vi "Impedance_Sweep_Freq.vi"(6 "Save Data?":bool, 8 "Freq Info":T1={"type"=1, "Number of\nTest Freqs"=128, "Start Freq"=100.0, "Stop Freq"=50000.0} {"Stop Freq" format="%#.4p"; "Start Freq" format="%#.4p"; "type" items=["Linear", "Logarithmic"]}, 9 "Saving Cluster":T2={"Experiment Title"="Experiment Title", "Save Path"=path "C:/Users/Human-MPI/Desktop/Temp", "File Name String"="TestStats", "Meta-Data Array"=[1.0]}, 10 "LCR Params":T4={"Rg_Vmon"=5000.0, "Rg_Imon"=5000.0, "ESL_Cal"=2.5e-07, "ESR_Cal"=0.0, "Cp_Cal"=0.0, "Rp_Cal"=1000000000.0, "UseCorrection"=TRUE, "R_Shunt"=100.0} {"R_Shunt" format="%#_6p"; "Rg_Vmon" format="%#_6p"; "Rg_Imon" format="%#_6p"; "ESL_Cal" format="%#_6p"; "ESR_Cal" format="%#_6p"; "Cp_Cal" format="%#_6p"; "Rp_Cal" format="%#_6p"}, 11 "Test Params Cluster":T3={"Test Freq. (Hz)"=0.0, "Output Signal Amplitude\nVolts Pk"=0.1, "Sampling Time (s)"=0.1, "Sampling Rate (Hz)"=2000000.0, "Output Channel"="PXI1Slot2/ao1", "Current Channel"="PXI1Slot2/ai1", "Voltage Channel"="PXI1Slot2/ai0", "Trigger Channel"="/PXI1Slot2/ao/StartTrigger", "Number of runs"=5} {"Output Signal Amplitude\nVolts Pk" format="%#_6p"; "Sampling Time (s)" format="%#_6p"; "Sampling Rate (Hz)" format="%#_6p"}) -> (0 "Single Run \nImpedance Cluster":T5={"|Z|"=nan, "Phase(Z)"=nan, "Re(Z)"=nan, "Imag(Z)"=nan, "Ls"=nan, "Cs"=nan, "Rp"=0.0, "Cp"=0.0} {"|Z|" format="%#_5p"; "Phase(Z)" format="%#_5p"; "Re(Z)" format="%#_5p"; "Imag(Z)" format="%#_5p"; "Ls" format="%#_5p"; "Cs" format="%#_5p"; "Rp" format="%#_5p"; "Cp" format="%#_5p"}, 1 "RealImag Graph":cluster{dbl[], dbl[]}[](graph), 2 "Mag Phase Graph":cluster{dbl[], dbl[]}[](graph), 3 "output cluster":T3={"Test Freq. (Hz)"=3243.3070866141734, "Output Signal Amplitude\nVolts Pk"=0.1, "Sampling Time (s)"=0.01, "Sampling Rate (Hz)"=250000.0, "Output Channel"="Dev3/ao0", "Current Channel"="Dev3/ai1", "Voltage Channel"="Dev3/ai0", "Trigger Channel"="/Dev3/ao/StartTrigger", "Number of runs"=5}, 4 "2D Compass":refnum<class "2D Plot Datatype.lvclass">[](xcontrol), 7 "Progress":i32(slide) scale=0.0..100.0)   [LabVIEW 2021]
uses:
  <vilib>/Math Plots/2D Math Plots/2D Compass/2D Compass XCtrl/2D Compass.xctl
  <vilib>/Analysis/1siggen.llb/Ramp Pattern by Samples.vi
  <vilib>/Analysis/baseanly.llb/Mean (DBL).vi
  <vilib>/Math Plots/2D Math Plots/2D Compass/2D Compass Datatype/Public/Plot Helper (Vector).vi
  <vilib>/Analysis/NI_AALBase.lvlib
  <vilib>/Math Plots/2D Math Plots/2D Compass/2D Compass Datatype/2D Compass Datatype.lvclass
panel:
  in  "Tab Control":enum32{"Inputs", "Outputs", "Additional Plots"}(tab)
  out "Test Number":i32=8
  out "Mean Mag":dbl format="%.4p"
  out "Mean Phase":dbl format="%0.2f"
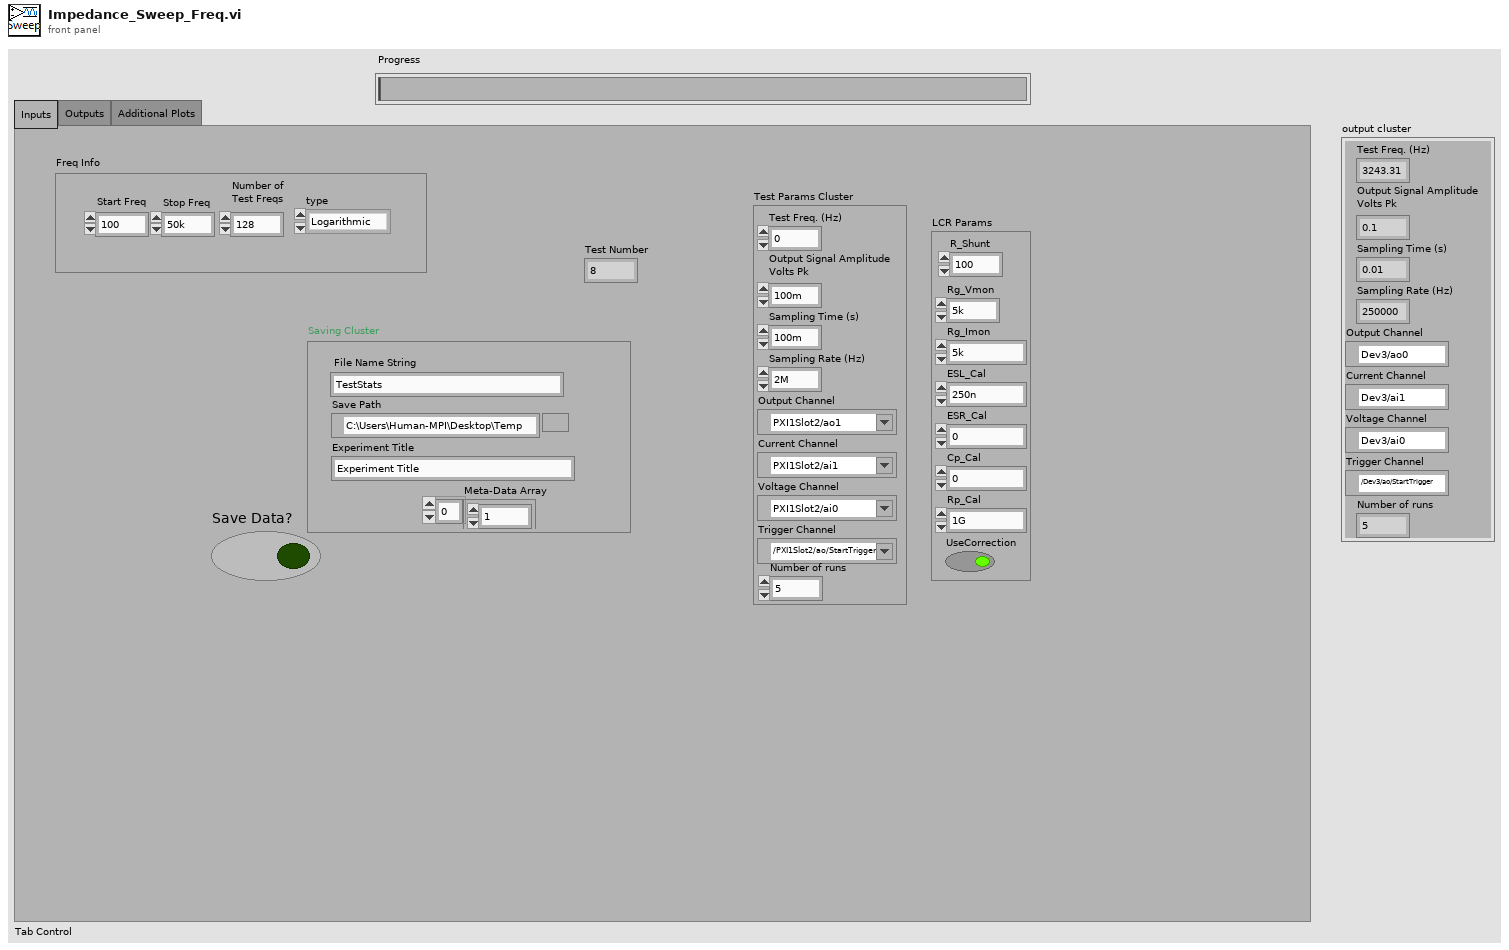
[diagram p1: front panel]
types:
  T1 = cluster{"type":u16, "Number of\nTest Freqs":i32, "Start Freq":dbl, "Stop Freq":dbl}
  T2 = cluster{"Experiment Title":string, "Save Path":path, "File Name String":string, "Meta-Data Array":dbl[]}
  T3 = cluster{"Test Freq. (Hz)":dbl, "Output Signal Amplitude\nVolts Pk":dbl, "Sampling Time (s)":dbl, "Sampling Rate (Hz)":dbl, "Output Channel":tag, "Current Channel":tag, "Voltage Channel":tag, "Trigger Channel":tag, "Number of runs":i32}
  T4 = cluster{"Rg_Vmon":dbl, "Rg_Imon":dbl, "ESL_Cal":dbl, "ESR_Cal":dbl, "Cp_Cal":dbl, "Rp_Cal":dbl, "UseCorrection":bool, "R_Shunt":dbl}
  T5 = cluster{"|Z|":dbl, "Phase(Z)":dbl, "Re(Z)":dbl, "Imag(Z)":dbl, "Ls":dbl, "Cs":dbl, "Rp":dbl, "Cp":dbl}
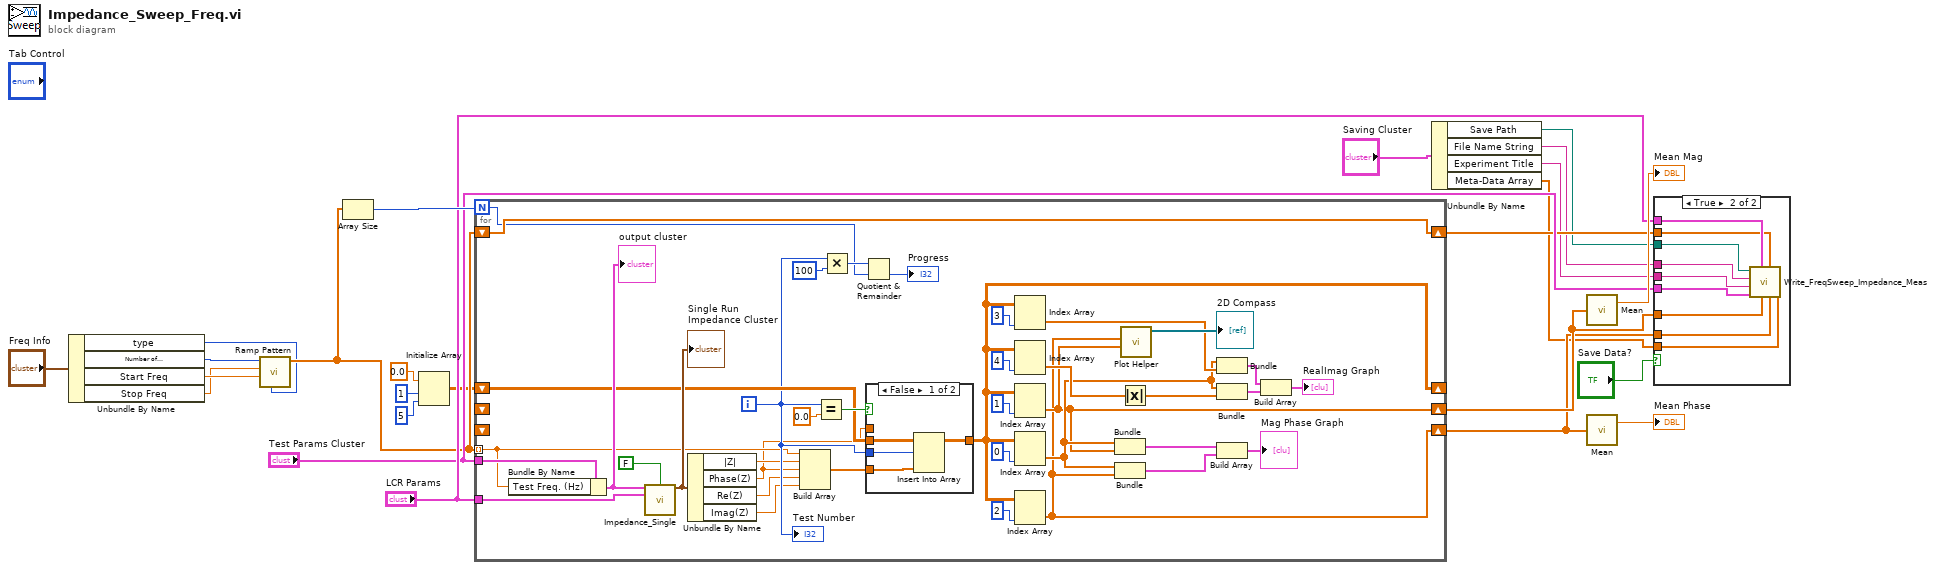
[diagram p0: block diagram]
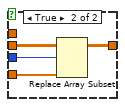
[diagram p3: hidden frame]
diagram:
  n1 = Unbundle By Name("Freq Info") -> ("type"=w7:u16, "Number of\nTest Freqs"=w8:i32, "Start Freq"=w6:dbl, "Stop Freq"=w5:dbl)
  n2 = call-poly <vilib>:"Ramp Pattern.vi"("type"=w7, "start"=w6, "end"=w5, "samples"=w8) -> ("Ramp Pattern"=w17:dbl[])  [unwired: 6 in, 1 out]
  n3 = Array Size(array=w17) -> (size(s)=w24:i32)
  n4 = Initialize Array(0.0 ("element"), 1 ("dimension size"), 5 ("dimension size")) -> (w14:dbl[][])
  n5 = for {
    N: w24 -> [w47]
    shift-right: [w56] -> w18
    shift-left: w17 -> [w56]
    tunnel: "Test Params Cluster" -> [w58]
    tunnel: "LCR Params" -> [w63]
    tunnel: w17 -> [w45] mode=indexing
    shift-right: [w25] -> _
    shift-left: w14 -> [w55]
    shift-right: [w27] -> w3
    shift-left: _ -> [_]
    shift-right: [w26] -> w2
    shift-left: _ -> [_]
    i -> [w46]
    n6 = Bundle By Name(cluster=w58, "Test Freq. (Hz)"=w45) -> (w57:T3)
    "output cluster" <- w57
    n7 = call "Impedance_Single.vi"("Test Params Cluster"=w57, "SaveFile?"=FALSE, "LCR Params"=w63) -> ("Mean Signal\nImpedance cluster"=w61:T5)  [unwired: 11 in, 1 out]
    "Single Run \nImpedance Cluster" <- w61
    n8 = Unbundle By Name(w61) -> ("|Z|"=w44:dbl, "Phase(Z)"=w43:dbl, "Re(Z)"=w42:dbl, "Imag(Z)"=w41:dbl)
    n9 = Build Array(w45, w44, w43, w42, w41) -> (w40:dbl[])
    n10 = Equal?(x=w46, y=0.0) -> (x = y?=w59:bool)
    n11 = Multiply(x=w46, y=100) -> (x*y=w48:i32)
    n12 = Quotient & Remainder(x=w48, y=w47) -> (floor(x/y)=→"Progress":i32)  [unwired: 1 out]
    n13 = case shown="False" w59 {
      tunnel: [w64 w71] -> w25
      tunnel: w43 -> [_ _]
      tunnel: w46 -> [w67 w70]
      tunnel: w55 -> [w66 w69]
      tunnel: w40 -> [w65 w68]
      frame False {
        n14 = Insert Into Array(array=w66, index (row)=w67, new element=w65) -> (w64:dbl[][])  [unwired: 1 in]
      }
      frame True {
        n15 = Replace Array Subset(array=w69, new element=w68, index (row)=w70) -> (w71:dbl[][])  [unwired: 1 in]
      }
    }
    n16 = Index Array(array=w25, index (col)=3 ("disabled index (col)")) -> (element=w33:dbl[])  [unwired: 1 in]
    n17 = Index Array(array=w25, index (col)=4 ("disabled index (col)")) -> (element=w34:dbl[])  [unwired: 1 in]
    n18 = Index Array(array=w25, index (col)=1 ("disabled index (col)")) -> (element=w27:dbl[])  [unwired: 1 in]
    n19 = Index Array(array=w25, index (col)=0 ("disabled index (col)")) -> (element=w32:dbl[])  [unwired: 1 in]
    n20 = Index Array(array=w25, index (col)=2 ("disabled index (col)")) -> (element=w26:dbl[])  [unwired: 1 in]
    n21 = Bundle(w32, w27) -> (w53:cluster{dbl[], dbl[]})  [unwired: 1 in]
    n22 = Bundle(w32, w26) -> (w29:cluster{dbl[], dbl[]})  [unwired: 1 in]
    n23 = Absolute Value(x=w34) -> (abs(x)=w51:dbl[])
    n24 = call-poly <vilib>:"Plot Helper.vi"("radius vector"=w27, "theta vector"=w26) -> ("2D Plot Class Obj Array out"=→"2D Compass":refnum<class "2D Plot Datatype.lvclass">[])  [unwired: 2 in, 7 out]
    n25 = Bundle(w32, w33) -> (w31:cluster{dbl[], dbl[]})  [unwired: 1 in]
    n26 = Bundle(w32, w51) -> (w52:cluster{dbl[], dbl[]})  [unwired: 1 in]
    n27 = Build Array(w53, w29) -> (→"Mag Phase Graph":cluster{dbl[], dbl[]}[])
    n28 = Build Array(w31, w52) -> (→"RealImag Graph":cluster{dbl[], dbl[]}[])
    "Test Number" <- w46
  }
  n29 = Unbundle By Name("Saving Cluster") -> ("Save Path"=w12:path, "File Name String"=w11:string, "Experiment Title"=w10:string, "Meta-Data Array"=w1:dbl[])
  n30 = call-poly <vilib>:"Mean.vi"("X"=w3) -> ("mean"=→"Mean Mag":dbl)  [unwired: 1 out]
  n31 = call-poly <vilib>:"Mean.vi"("X"=w2) -> ("mean"=→"Mean Phase":dbl)  [unwired: 1 out]
  n32 = case shown="True" "Save Data?" {
    tunnel: "LCR Params" -> [_ w80]
    tunnel: w12 -> [_ w79]
    tunnel: w11 -> [_ w78]
    tunnel: w10 -> [_ w77]
    tunnel: "Test Params Cluster" -> [_ w76]
    tunnel: w18 -> [_ w75]
    tunnel: w3 -> [_ w74]
    tunnel: w2 -> [_ w73]
    tunnel: w1 -> [_ w72]
    frame False {
    }
    frame True {
      n33 = call "Write_FreqSweep_Impedance_Meas.vi"("Meta-Data Array"=w72, "Z_Phase_Vec"=w73, "Freq Vector"=w75, "|Z| Vector"=w74, "Compensation and Gain"=w80, "Test Params Cluster"=w76, "Experiment Title"=w77, "File Name String"=w78, "Path"=w79) -> ()  [unwired: 3 in]
    }
  }
